vi "Add Error.vi"(8 "error in (no error)":errorcluster, 11 "Output cluster":T1) -> (0 "error out":errorcluster)   [LabVIEW 2021]
uses:
  Type defs/Queues.ctl
  Type defs/Message cluster.ctl
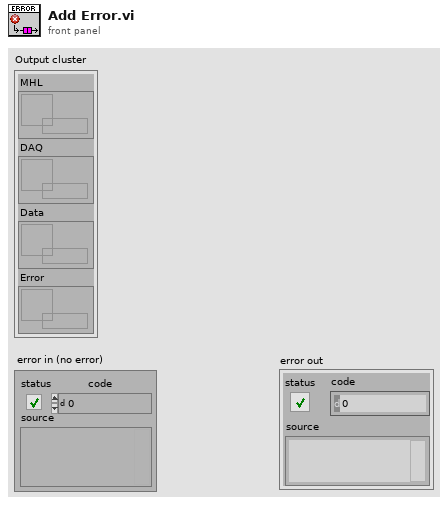
[diagram p1: front panel]
types:
  T1 = typedef "Queues.ctl" = cluster{"MHL":refnum<queue>, "DAQ":refnum<queue>, "Data":refnum<queue>, "Error":refnum<queue>}
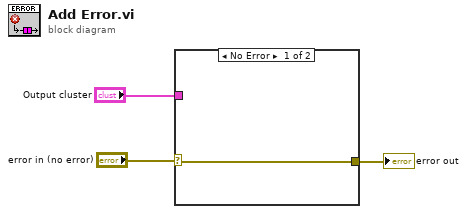
[diagram p0: block diagram]
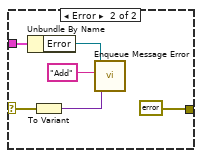
[diagram p2: hidden frame]
diagram:
  n1 = case shown="No Error" "error in (no error)" {
    selector: "error in (no error)" -> [w4 w9]
    tunnel: "Output cluster" -> [_ w10]
    tunnel: [w4 errorcluster {"status"=FALSE, "code"=0, "source"=""} ("error IO")] -> w1
    frame No Error {
    }
    frame Error {
      n2 = Unbundle By Name(w10) -> ("Error"=w8:refnum<queue>)
      n3 = To Variant(anything=w9) -> (Variant=w6:variant)
      n4 = call "Enqueue Message Error.vi"("Data"=w6, "Message"="Add", "queue in"=w8) -> ()  [unwired: 7 in, 2 out]
    }
  }
  "error out" <- w1
